vi "Order Power Spectrum.vi"() -> ()   [LabVIEW 2026, in "SoundVib_MCM Examples.lvlib"]
doc: "This VI demonstrates how to compute an order power spectrum with averaging. This VI uses DAQmx VIs to acquire sound or vibration signals and an analog tachometer signal and displays the order power spectrum continuously. \n\n<B>INSTRUCTIONS</B>:\n1. On the <B>DAQ Configurations</B> page, specify the device and channel configurations, time settings, and tachometer channel information.\n2. On the <B>Order Power Spectrum</B> page, specify the <B>window type</B>, <B>block size</B> or <B>order resolution</B>, and <B>averaging parameters</B> for power in band computation. \n3. Run the VI.\n\n<B>VIs USED IN THIS EXAMPLE</B>:\n1. OAT Analog Tacho Process.vi\n2. OAT Convert to Even Angle Signal.vi\n3. OAT Order Power Spectrum.vi\n4. SVFA Power in Band.vi"
uses:
  Program Files/NI/LVAddons/nisvt/1/examples/Order Analysis/SoundVib_MCM Examples.lvlib
  <vilib>/addons/Sound and Vibration/svt_DAQmx/Configuration XControl/SVX NI-DAQmx AI Configuration XControl.xctl
  <vilib>/DAQmx/read.llb/DAQmx Read (Analog 1D Wfm NChan NSamp).vi
  <vilib>/DAQmx/miscellaneous.llb/DAQmx Fill In Error Info.vi
  <vilib>/addons/Sound and Vibration/Order Analysis/Tach Process/OAT Analog Tacho Process (1 Tacho).vi
  <vilib>/addons/Sound and Vibration/Order Analysis/Resample Order Tracking/OAT Convert to Even Angle Signal (N Channels).vi
  <vilib>/addons/Sound and Vibration/Order Analysis/Resample Order Tracking/OAT Order Power Spectrum (N Channels).vi
  <vilib>/addons/Sound and Vibration/Order Analysis/Tach Process/SoundVib_TachProcess.lvlib
  <vilib>/addons/Sound and Vibration/Order Analysis/Resample Order Tracking/SoundVib_OrderTracking.lvlib
  <resource>/objmgr/daqmx.rc
panel:
  in  "stop":bool
  in  "Tab Control":T1(tab)
  in  "DAQmx AI Config":refnum<k21>(xcontrol)
  out "Speed profile":cluster{"time [s]":dbl[], "speed [RPM]":dbl[]}(graph)
  out "Acquired waveform":waveform(dbl)[](graph)
  out "actual max order":dbl
  in  "restart averaging (F)":bool
  in  "averaging parameters":T2={"averaging mode"=enum."RMS averaging", "weighting mode"=enum."Exponential", "number of averages"=10, "linear mode"=enum."One shot"} {"number of averages" min=1 step=1}
  in  "window type":u32(ring) items=["None"=0, "Hanning"=1, "Hamming"=2, "Blackman-Harris"=3, "Exact Blackman"=4, "Blackman"=5, "Flat Top"=6, "4 Term B-Harris"=7, "7 Term B-Harris"=8, "Low Sidelobe"=9, "Gaussian"=62]
  in  "dB on? (T)":bool=TRUE
  out "order power spectra":T3(graph)
  # "Select Help»Show Context Help and move the cursor over the VI  icon for more information."
  # "You can specify Channel Type = Voltage (V) for most tachometers. For this example, you must select Reference Type = Analog Tachometer and select a Tachometer Channel = channel in Channel Table."
  # "General Settings"
  # "Averaging Settings"
  # "Power in Band"
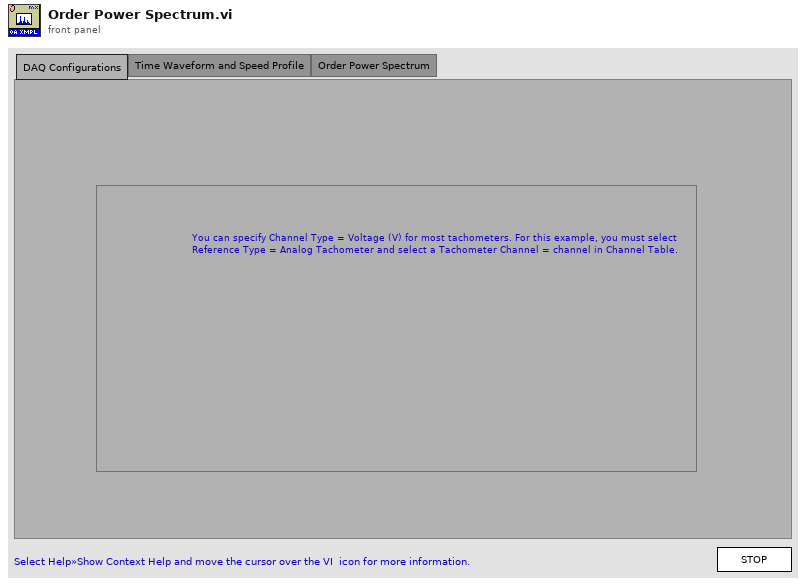
[diagram p1: front panel]
types:
  T1 = enum32{"DAQ Configurations", "Time Waveform and Speed Profile", "Order Power Spectrum"}
  T2 = cluster{"averaging mode":enum16{"No averaging", "Vector averaging", "RMS averaging", "Peak hold"}, "weighting mode":enum16{"Linear", "Exponential"}, "number of averages":u32, "linear mode":enum16{"One shot", "Auto restart"}}
  T3 = cluster{"order 0":dbl, "delta order":dbl, "magnitude":dbl[]}[]
  T4 = typedef "SoundVib_TachProcess.lvlib/speed profile.ctl" = cluster{"time [s]":dbl[], "speed [RPM]":dbl[]}
  T5 = typedef "svc_Resampled Channel Info.ctl" = cluster{"channel name":string, "description":string, " channel info":T6}
  T6 = typedef "svc_Channel Info.ctl" = cluster{"sensor sensitivity":dbl, "engineering units":T7, "dB reference":dbl, "custom label":string, "weighting filter":T8, "pregain":dbl}
  T7 = typedef "svc_Engineering Units Text Ring.ctl" = u16
  T8 = typedef "svc_Weighting Filter Text Ring.ctl" = u16
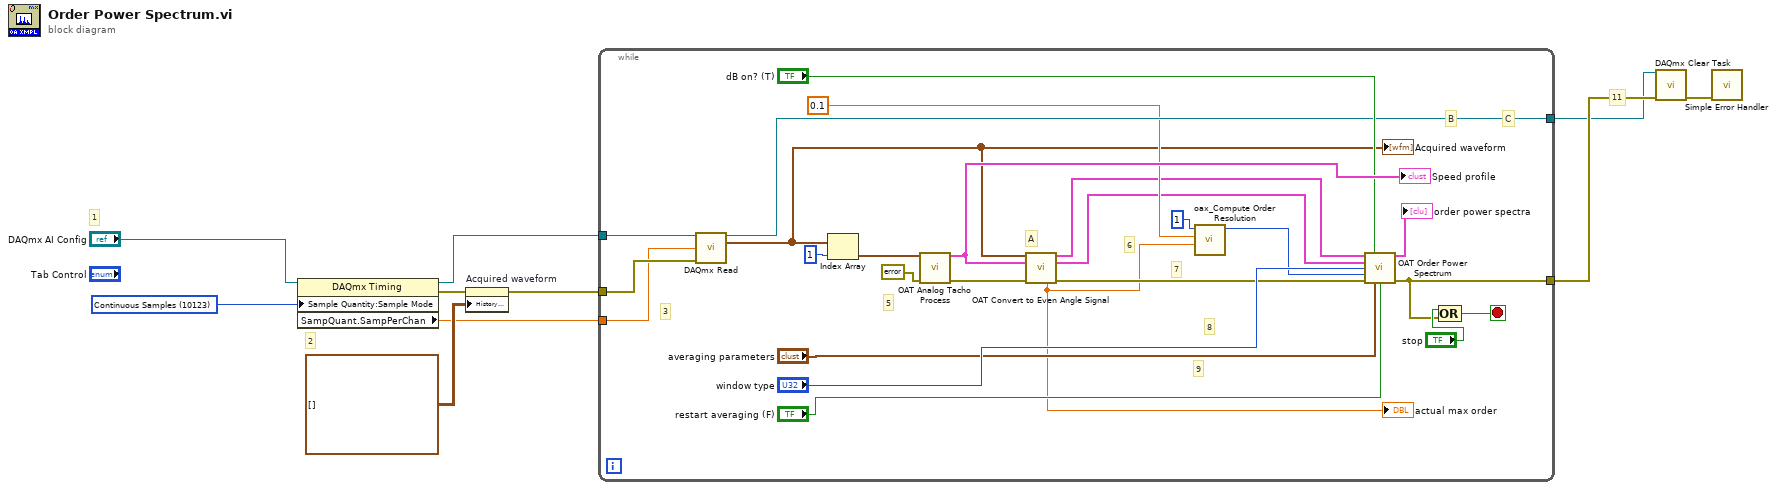
[diagram p0: block diagram]
diagram:
  w6 = 10123 items=["Finite Samples"=10178, "Continuous Samples"=10123, "Hardware Timed Single Point"=12522] ("SampQuant.SampMode")
  # "2"
  # "11"
  # "1"
  n1 = property class="DAQmx Timing"(reference="DAQmx AI Config", "Sample Quantity:Sample Mode"=w6) -> (reference out=w2:refnum<k21>, error out=w4:errorcluster, "SampQuant.SampPerChan"=w3:dbl)  [unwired: 1 in]
  n2 = property on="Acquired waveform" class="WFChart (strict)"(error in=w4, "History Data"=waveform(dbl)[][] []) -> (error out=w5:errorcluster)  [unwired: 1 in, 1 out]
  n3 = while {
    tunnel: [w28] -> w8
    tunnel: [w29] -> w10
    tunnel: w5 -> [w18]
    tunnel: w3 -> [w17]
    tunnel: w2 -> [w16]
    stop <- w35 stop-if-true
    # "C"
    # "B"
    # "A"
    # "9"
    # "8"
    # "7"
    # "6"
    # "5"
    # "3"
    n4 = call-poly <vilib>:"DAQmx Read.vi"("task/channels in"=w16, "number of samples per channel"=w17, "error in"=w18) -> ("task out"=w28:refnum<k21>, "data"=w14:waveform(dbl)[])  [unwired: 10 in, 1 out]
    "Acquired waveform" <- w14
    n5 = Index Array(array=w14, index=1) -> (element=w13:waveform(dbl))
    n6 = call-poly <vilib>:"OAT Analog Tacho Process.vi"("analog tacho signal"=w13, "error in (no error)"=errorcluster {"status"=TRUE, "code"=-21414, "source"="<ERR>The DAQ config input is invalid. Select one tacho channel and at least one sound or vibration channel in the configuration control. "} ("t")) -> ("speed profile"=w33:T4, "error out"=w26:errorcluster)  [unwired: 9 in, 3 out]
    "Speed profile" <- w33
    n7 = call-poly <vilib>:"OAT Convert to Even Angle Signal.vi"("scaled signals [EU]"=w14, "speed profile"=w33, "error in (no error)"=w26) -> ("even-angle signals"=w23:cluster{"r0":dbl, "dr":dbl, "Y":dbl[]}[], "even-angle channel info"=w21:T5[], "actual max order"=w19:dbl, "error out"=w24:errorcluster)  [unwired: 8 in, 1 out]
    "actual max order" <- w19
    n8 = call <vilib>:"oax_Compute Order Resolution.vi"("actual max order"=w19, "order resolution"=0.1, "block size"=1) -> ("block size out"=w22:i32)  [unwired: 7 in, 1 out]
    n9 = call-poly <vilib>:"OAT Order Power Spectrum.vi"("even-angle signals"=w23, "dB on? (T)"="dB on? (T)", "even-angle channel info"=w21, "window"="window type", "block size"=w22, "error in (no error)"=w24, "averaging parameters"="averaging parameters", "restart averaging? (F)"="restart averaging (F)") -> ("order power spectra"=→"order power spectra":T3, "error out"=w29:errorcluster)  [unwired: 1 in, 5 out]
    n10 = Compound Arithmetic op=OR("stop", w29) -> (w35:bool)
  }
  n11 = call <vilib>:"DAQmx Clear Task.vi"("task in"=w8, "error in"=w10) -> ("error out"=w9:errorcluster)  [unwired: 13 in]
  n12 = call <vilib>:"Simple Error Handler.vi"("error in (no error)"=w9) -> ()  [unwired: 4 in, 5 out]
